vi "P1_OpenVIReference.vi"(11 "Inputs":string[](array[string])) -> (2 "Output/Failure":string, 3 "CLI Process Return Code":i32)   [LabVIEW 2026]
doc: "Slice 1.1 probe: Open VI Reference, then Close Reference."
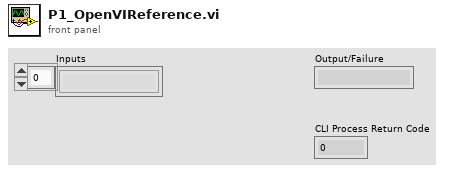
[diagram p1: front panel]
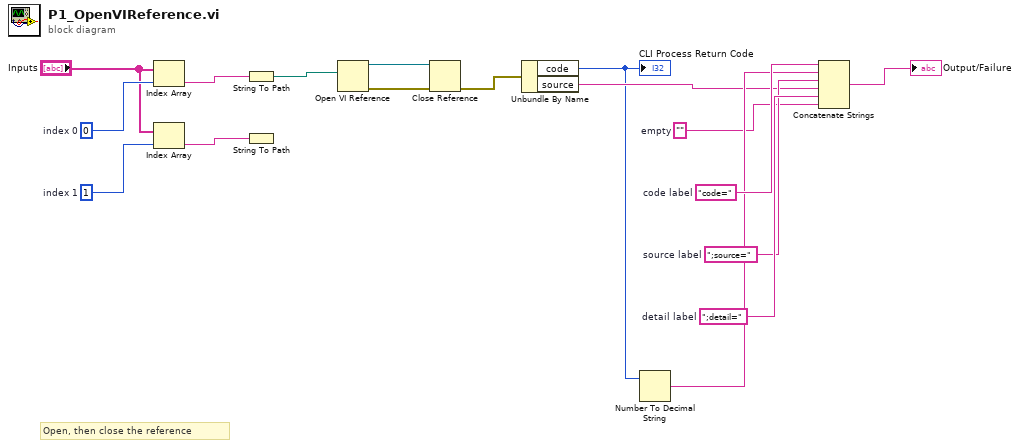
[diagram p0: block diagram]
diagram:
  w16 = ";detail="  # detail label
  w15 = ";source="  # source label
  w14 = "code="  # code label
  w7 = ""  # empty
  w3 = 1  # index 1
  w2 = 0  # index 0
  # "Open, then close the reference"
  n1 = Index Array(array="Inputs", index=w2) -> (element=w4:string)
  n2 = Index Array(array="Inputs", index=w3) -> (element=w5:string)
  n3 = String To Path(string=w4) -> (path=w6:path)
  n4 = String To Path(string=w5) -> ()  [unwired: 1 out]
  n5 = Open VI Reference(vi path=w6) -> (vi reference=w8:refnum<vi>, error out=w9:errorcluster)  [unwired: 5 in]
  n6 = Close Reference(reference=w8, error in (no error)=w9) -> (error out=w10:errorcluster)
  n7 = Unbundle By Name(w10) -> ("code"=w11:i32, "source"=w12:string)
  "CLI Process Return Code" <- w11
  n8 = Number To Decimal String(number=w11) -> (decimal integer string=w13:string)  [unwired: 1 in]
  n9 = Concatenate Strings(w14, w13, w15, w12, w16, w7) -> (→"Output/Failure":string)
